vi "Binary to KLB(64-bit)Multiple Files.vi"() -> ()   [LabVIEW 2013]
uses:
  File IO/KLB/VIs/Type Defs/KLB Settings Cluster.ctl
  File IO/KLB/VIs/Type Defs/KLB # of CPUs enum.ctl
  File IO/KLB/VIs/Type Defs/KLB compression type enum.ctl
  Common/Timing/Timestamp with error IO.vi
  <vilib>/vision/Image Controls.llb/IMAQ Image.ctl
  File IO/KLB/KLB.lvlib
panel:
  out "Numeric":i32
  out "String":string
  out "size(s)":i32
  out "Processing File":i32=1
  in  "KLB Settings":T1={"Logical Cores"=enum."CPU 75%", "pixelSize (um)"=[1.0, 1.0, 1.0, 1.0, 1.0], "blockSize"=[384, 192, 1, 1, 1], "compressionType"=enum."BZip2", "metadata"=""} {"pixelSize (um)" min=0.01 max=10 step=0.01 format="%.2f"}
  out "Image":T4(plugin-control)
  out "KLB Conversion Time (ms)":u32
  out "Image/Sector Size(bytes)":i64=165406205104
  in  "stop":bool
  out "Progress":u64(slide)=174919 max=5098 scale=0.0..56939.0
  out "Partial images in file?":bool
  out "# of Images":u32=174919
  out "error IO":errorcluster
  out "Height":u32=788
  out "Width":u32=1200
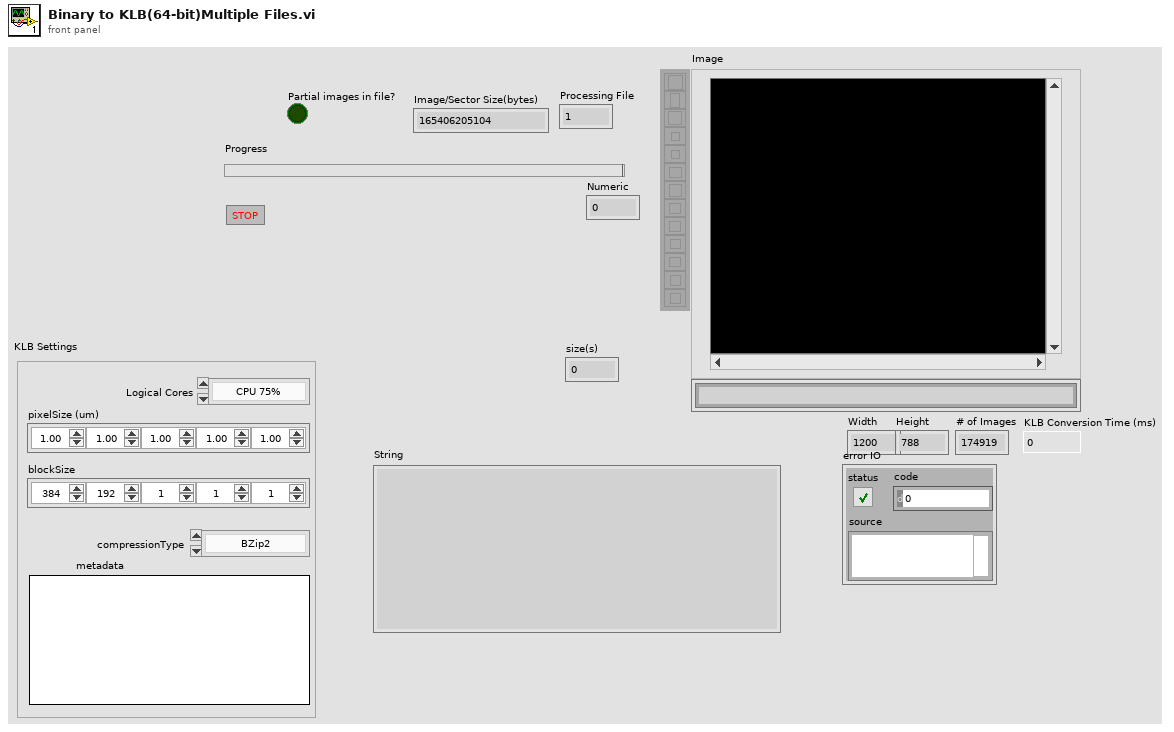
[diagram p1: front panel]
types:
  T1 = typedef "KLB.lvlib/KLB Settings Cluster.ctl" = cluster{"Logical Cores":T2, "pixelSize (um)":sgl[], "blockSize":u32[], "compressionType":T3, "metadata":string}
  T2 = typedef "KLB.lvlib/KLB # of CPUs enum.ctl" = enum16{"CPU 25%", "CPU 50%", "CPU 75%", "CPU All but 1", "1", "4", "8", "16"}
  T3 = typedef "KLB.lvlib/KLB compression type enum.ctl" = enum8{"Uncompressed", "BZip2"}
  T4 = typedef "IMAQ Image.ctl" = refnum<image>
  T5 = typedef "Mask ROI Cluster.ctl" = cluster{"left annulus":T6, "right annulus":T6, "Threshold Range":cluster{"Lower value":dbl, "Upper value":dbl}, "[Avg BG]":u8[], "Number of Sectors":u8, "Left ROI":T7, "Right ROI":T7, "Left Start Angle Duty Cycle":fxp<+,8,0>, "Left End Angle Duty Cycle":fxp<+,8,0>, "Right End Angle Duty Cycle":fxp<+,8,0>, "Right Start Angle Duty Cycle":fxp<+,8,0>, "[Sector ROIs]":T7[], "Consecutive Sector Threshold":u8}
  T6 = typedef "IMAQ Circle" = cluster{"Center X":i32, "Center Y":i32, "Inner Radius":i32, "Outer Radius":i32, "Start Angle":dbl, "End Angle":dbl}
  T7 = typedef "ROI Descriptor" = cluster{"Global Rectangle":i32[], "Contours":cluster{"ID":enum32{"External", "Internal"}, "Type":u32, "Coordinates":i32[]}[]}
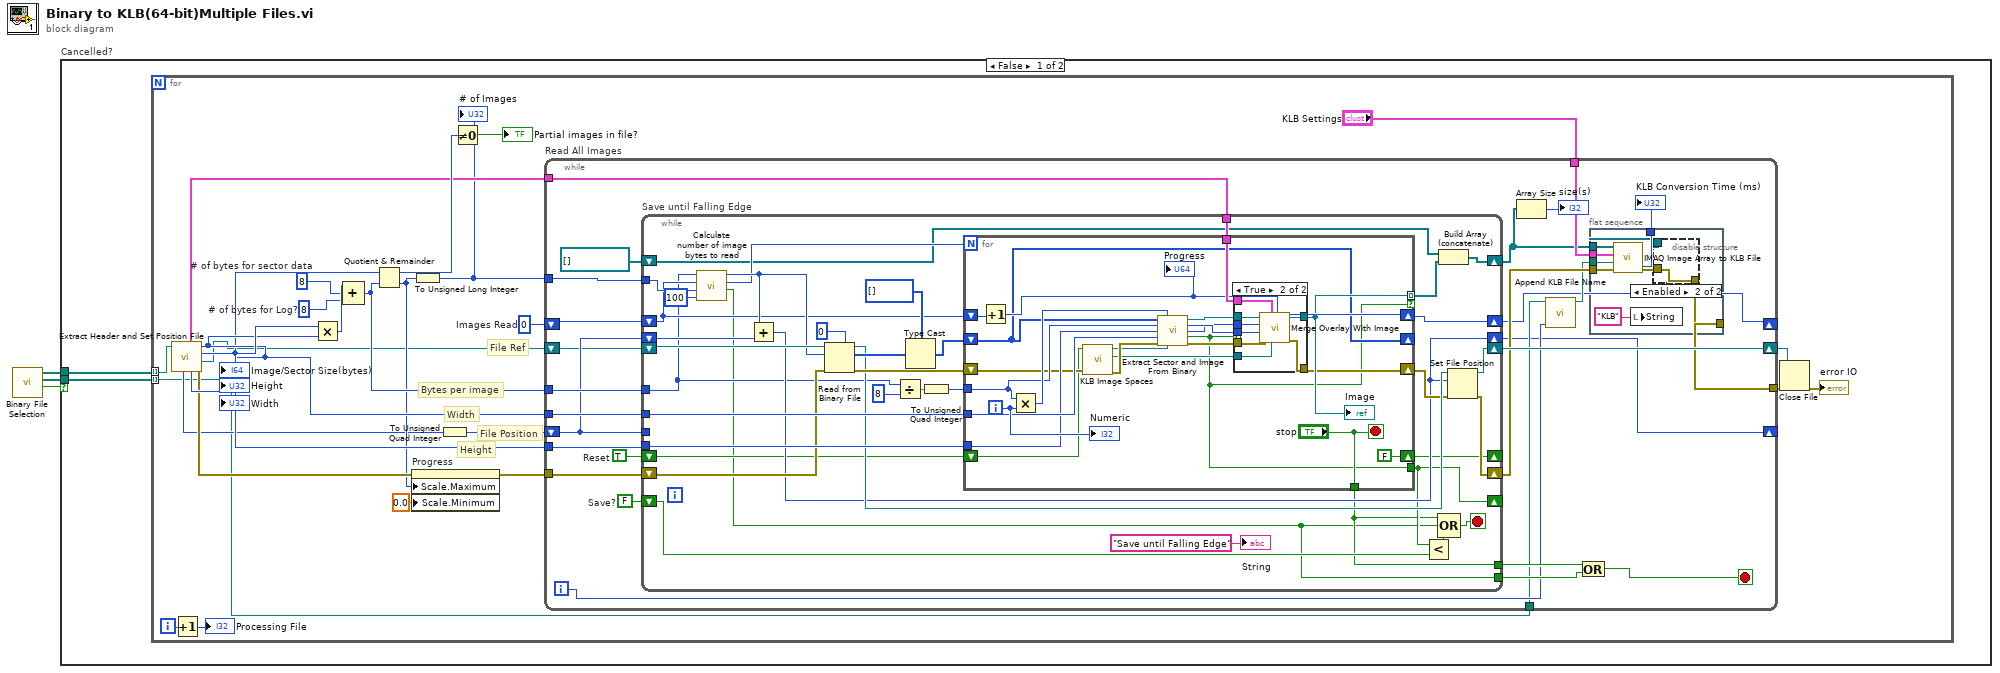
[diagram p0: block diagram]
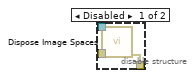
[diagram p2: hidden frame]
diagram:
  n1 = call "Binary File Selection.vi"() -> ("cancelled"=w3:bool, "klb paths"=w1:path[], "selected paths"=w2:path[])  [unwired: 9 in]
  n2 = case "Cancelled?" shown="False" w3 {
    tunnel: w2 -> [w5 _]
    tunnel: w1 -> [w4 _]
    frame False {
      n3 = for {
        tunnel: w5 -> [w11] mode=indexing
        tunnel: w4 -> [w10] mode=indexing
        i -> [w7]
        w8 = u32 0  # Images Read
        w13 = u32 8  # # of bytes for Log?
        w26 = u32 8  # # of bytes for sector data
        # "File Position"
        # "Height"
        # "Width"
        # "Bytes per image"
        # "File Ref"
        n4 = call "Extract Header and Set Position File.vi"("Binary File"=w11) -> ("error out"=w21:errorcluster, "refnum out"=w16:refnum<file>, "Height"=w24:u32, "Width"=w23:u32, "Image/Sector Size(bytes)"=w22:i64, "Mask ROI Out"=w17:T5, "Header Size"=w19:i32)  [unwired: 4 in]
        "Width" <- w23
        "Height" <- w24
        "Image/Sector Size(bytes)" <- w22
        n5 = Increment(x=w7) -> (x+1=→"Processing File":i32)
        n6 = Multiply(x=w24, y=w23) -> (x*y=w27:u32)
        n7 = Compound Arithmetic op=ADD(w27, w26, w13) -> (w25:u32)
        n8 = Quotient & Remainder(x=w22, y=w25) -> (x-y*floor(x/y)=w31:i64, floor(x/y)=w20:i64)
        n9 = property on="Progress" class="Slide (strict)"(error in=w21, "Scale.Maximum"=w20, "Scale.Minimum"=0.0 ("Data Entry Limits:Minimum")) -> (error out=w29:errorcluster)  [unwired: 1 in, 1 out]
        n10 = To Unsigned Long Integer(number=w20) -> (unsigned 32bit integer=w15:u32)
        "# of Images" <- w15
        n11 = To Unsigned Quad Integer(1:w19) -> (0:w18:u64)
        n12 = Not Equal To 0?(x=w31) -> (x != 0?=→"Partial images in file?":bool)
        n13 = while "Read All Images" {
          tunnel: w29 -> [w58]
          tunnel: w25 -> [w57]
          tunnel: w24 -> [w56]
          tunnel: w23 -> [w55]
          tunnel: w17 -> [w53]
          tunnel: w15 -> [w51]
          tunnel: "KLB Settings" -> [w48]
          tunnel: w10 -> [w39]
          tunnel: [w45] -> w9
          shift-right: [w59] -> w30
          shift-left: w16 -> [w52]
          shift-right: [w36] -> _
          shift-left: w8 -> [w37]
          shift-right: [w35] -> _
          shift-left: w18 -> [w54]
          i -> [w40]
          stop <- w41 stop-if-true
          w44 = FALSE  # Save?
          w47 = TRUE  # Reset
          n14 = while "Save until Falling Edge" {
            tunnel: w55 -> [w109]
            tunnel: w56 -> [w108]
            shift-right: [w101] -> w46
            shift-left: w58 -> [w106]
            shift-right: [w99] -> w59
            shift-left: w52 -> [w107]
            tunnel: w57 -> [w87]
            tunnel: w54 -> [_]
            shift-right: [w91] -> w36
            shift-left: w37 -> [w92]
            tunnel: w51 -> [w98]
            shift-right: [w89] -> w35
            shift-left: w54 -> [w96]
            tunnel: w53 -> [w88]
            shift-right: [w82] -> w34
            shift-left: T4[] [] -> [w81]
            shift-right: [w79] -> _
            shift-left: w47 -> [w80]
            shift-right: [w78] -> _
            shift-left: w44 -> [w77]
            tunnel: [w75] -> w43
            tunnel: [w74] -> w42
            stop <- w97 stop-if-true
            n15 = call "Calculate number of image bytes to read.vi"("Images per Chunk"=u32 100, "# of total images"=w98, "Total Images Read"=w92, "# of bytes per image"=w87) -> ("All Images Read?"=w74:bool, "# of Images Read"=w93:u32, "# of bytes to read"=w95:u64)  [unwired: 5 in]
            n16 = Add(x=w95, y=w96) -> (x+y=w89:u64)
            n17 = Read from Binary File(5:u8 0, 8:w106, 10:w95, 11:w107) -> (0:w105:errorcluster, 2:w103:u8[], 3:w100:refnum<file>)  [unwired: 2 in, 1 out]
            n18 = Divide(x=w87, y=u32 8) -> (x/y=w85:dbl)
            n19 = Type Cast(type=u64[] [], x=w103) -> (*(type *) &x=w94:u64[])
            n20 = To Unsigned Quad Integer(1:w85) -> (0:w84:u64)
            n21 = for {
              N: w93 -> [_]
              tunnel: w109 -> [w130]
              tunnel: w108 -> [w129]
              shift-right: [w122] -> w91
              shift-left: w92 -> [w128]
              shift-right: [w119] -> w90
              shift-left: w105 -> [w116]
              tunnel: ["stop"] -> w75
              tunnel: w88 -> [w125]
              tunnel: w84 -> [w121]
              tunnel: [w120] -> w83 mode=indexing if=w110
              shift-right: [w117] -> _
              shift-left: w94 -> [w117]
              shift-right: [FALSE ("Reset")] -> w79
              shift-left: w80 -> [w112]
              tunnel: [w110] -> w78
              i -> [w132]
              stop <- "stop" stop-if-true
              n22 = Increment(x=w128) -> (x+1=w122:u32)
              "Progress" <- w122
              n23 = Multiply(x=w121, y=w132) -> (x*y=w131:u64)
              n24 = call "KLB Image Spaces.vi"("error in (no error)"=w116, "Reset?"=w112) -> ("error out"=w115:errorcluster, "RGB Image"=w113:T4, "U8 Image"=w114:T4)  [unwired: 7 in]
              n25 = call "Extract Sector and Image From Binary.vi"("Binary Data(u64)"=w117, "Start Index"=w131, "# of u64 per image"=w121, "Height"=w129, "Width"=w130, "error in (no error)"=w115, "Image Destination"=w114) -> ("Image Out"=w126:T4, "Left Sector"=w124:u16, "Right Sector"=w123:u16, "Log?"=w110:bool, "error out"=w118:errorcluster)  [unwired: 4 in]
              n26 = case shown="True" w110 {
                tunnel: w126 -> [w134 w142]
                tunnel: w125 -> [_ w141]
                tunnel: w124 -> [_ w140]
                tunnel: w123 -> [_ w139]
                tunnel: [w134 w138] -> w120
                tunnel: [w133 w137] -> w119
                tunnel: w118 -> [w133 w136]
                tunnel: w113 -> [_ w135]
                frame False {
                }
                frame True {
                  n27 = call "Merge Overlay With Image.vi"("Image RGB"=w135, "ROI Cluster"=w141, "Error in"=w136, "Left Edge"=w140, "Right Edge"=w139, "Image In"=w142) -> ("error out"=w137:errorcluster, "Image Out"=w138:T4)  [unwired: 4 in]
                }
              }
              "Image" <- w120
              "Numeric" <- w132
            }
            n28 = Less?(x=w78, y=w77) -> (x < y?=w76:bool)
            n29 = Compound Arithmetic op=OR(w75, w74, w76) -> (w97:bool)
            n30 = Build Array (concatenate)(w81, w83) -> (w82:T4[])
            n31 = Set File Position(offset (in bytes) (0)=w89, refnum=w100, error in=w90) -> (refnum out=w99:refnum<file>, error out=w101:errorcluster)  [unwired: 1 in]
            "String" <- "Save until Falling Edge" ("String")
          }
          n32 = Array Size(array=w34) -> (size(s)=→"size(s)":i32)
          n33 = call "Append KLB File Name.vi"("Iteration"=w40, "Path In"=w39) -> ("Path Out"=w38:path)  [unwired: 9 in]
          n34 = Compound Arithmetic op=OR(w43, w42) -> (w41:bool)
          n35 = flat-sequence {
            tunnel: [w67] -> w50
            tunnel: w48 -> [w66]
            tunnel: w46 -> [w64]
            tunnel: [w63] -> w45
            tunnel: w38 -> [w62]
            tunnel: w34 -> [w61]
            frame #0 {
              n36 = call "IMAQ Image Array to KLB File.vi"("error in (no error)"=w64, "path"=w62, "KLB Settings"=w66, "Images to Compress"=w61) -> ("error out"=w65:errorcluster, "elapsed (ms)"=w67:u32)  [unwired: 6 in]
              n37 = local write "String"("KLB" ("String")) -> ()
              n38 = disable-structure shown="Enabled" {
                disable-tunnel: w65 -> [w70 w71]
                disable-tunnel: [w69 w71] -> w63
                disable-tunnel: w61 -> [w68 _]
                frame Disabled {
                  n39 = call "Dispose Image Spaces.vi"("error in (no error)"=w70, "[Images]"=w68) -> ("error out"=w69:errorcluster)  [unwired: 9 in]
                }
                frame Enabled {
                }
              }
            }
          }
          "KLB Conversion Time (ms)" <- w50
        }
        n40 = Close File(refnum=w30, error in=w9) -> (error out=→"error IO":errorcluster)  [unwired: 1 out]
      }
    }
    frame True {
    }
  }
